vi "Scale_4to20mA.vi"(0 "Current_mA":dbl=4.0, 5 "High_Limit_Pct":dbl=80.0, 7 "Low_Limit_Pct":dbl=20.0, 11 "error in":errorcluster) -> (4 "Scaled_Pct":dbl, 6 "High_Alarm":bool, 8 "Low_Alarm":bool, 15 "error out":errorcluster)   [LabVIEW 2026]
doc: "4-20 mA current input scaled to 0-100 % engineering units, with high/low limit alarms.\nScaled_Pct = (Current_mA - 4.0) / 16.0 * 100.0\nHigh_Alarm = Scaled_Pct > High_Limit_Pct. Low_Alarm = Scaled_Pct < Low_Limit_Pct.\nThe calculation runs only when error in carries no error. Otherwise outputs are 0 / False and the error passes through."
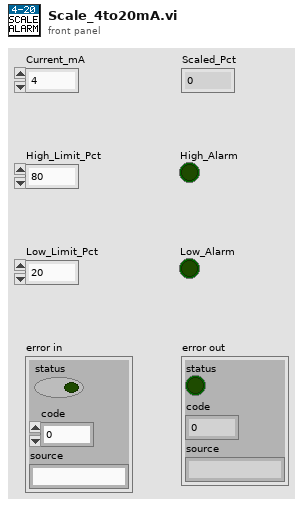
[diagram p1: front panel]
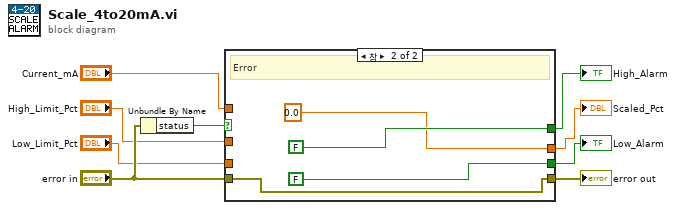
[diagram p0: block diagram]
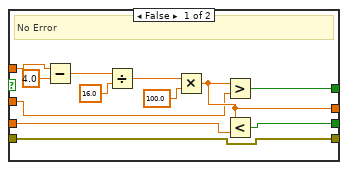
[diagram p2: hidden frame]
diagram:
  n1 = Unbundle By Name("error in") -> ("status"=w9:bool)
  n2 = case shown="참" w9 {
    tunnel: "Current_mA" -> [w10 _]
    tunnel: "High_Limit_Pct" -> [w11 _]
    tunnel: "Low_Limit_Pct" -> [w12 _]
    tunnel: "error in" -> [w13 w22]
    tunnel: [w13 w22] -> w8
    tunnel: [w19 0.0] -> w5
    tunnel: [w20 FALSE] -> w6
    tunnel: [w21 FALSE] -> w7
    frame False {
      # "No Error"
      n3 = Subtract(x=w10, y=4.0) -> (x-y=w17:dbl)
      n4 = Divide(x=w17, y=16.0) -> (x/y=w18:dbl)
      n5 = Multiply(x=w18, y=100.0) -> (x*y=w19:dbl)
      n6 = Greater?(x=w19, y=w11) -> (0:w20:bool)
      n7 = Less?(x=w19, y=w12) -> (x < y?=w21:bool)
    }
    frame True {
      # "Error"
    }
  }
  "Scaled_Pct" <- w5
  "High_Alarm" <- w6
  "Low_Alarm" <- w7
  "error out" <- w8
